vi "analyze cpu.vi"(8 "error in (no error)":errorcluster, 10 "offset (0)":i64, 11 "file path":path) -> (0 "error out":errorcluster, 2 "cpu load stats":T1, 3 "data":dbl[](array[numeric]))   [LabVIEW 2014]
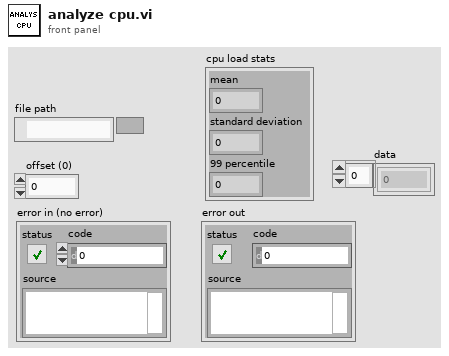
[diagram p1: front panel]
types:
  T1 = cluster{"mean":dbl, "standard deviation":dbl, "99 percentile":dbl}
  T2 = cluster{"mean":dbl, "standard deviation":dbl, "calculated percentiles":dbl[], "slope":dbl, "max":dbl}
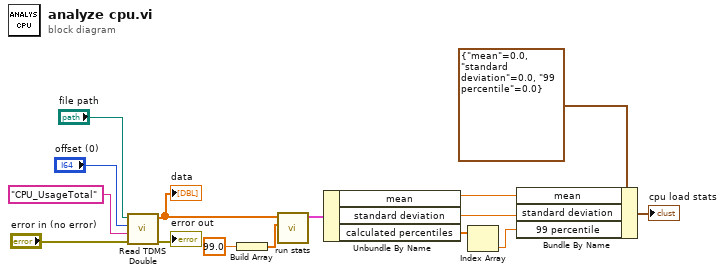
[diagram p0: block diagram]
diagram:
  n1 = call "Read TDMS Double.vi"("error in (no error)"="error in (no error)", "channel name(s) in"="CPU_UsageTotal", "offset (0)"="offset (0)", "file path"="file path") -> ("error out"=→"error out":errorcluster, "Data"=w8:dbl[])  [unwired: 6 in]
  "data" <- w8
  n2 = Build Array(99.0 ("p")) -> (w9:dbl[])
  n3 = call "run stats.vi"("percentiles"=w9, "Data"=w8) -> ("stats out"=w7:T2)  [unwired: 9 in]
  n4 = Unbundle By Name(w7) -> ("mean"=w5:dbl, "standard deviation"=w4:dbl, "calculated percentiles"=w3:dbl[])
  n5 = Index Array(array=w3) -> (element=w2:dbl)  [unwired: 1 in]
  n6 = Bundle By Name(cluster=T1 {"mean"=0.0, "standard deviation"=0.0, "99 percentile"=0.0} ("cpu load stats"), "mean"=w5, "standard deviation"=w4, "99 percentile"=w2) -> (→"cpu load stats":T1)
